vi "Prcess Data.vi"(8 "error in (no error)":errorcluster, 9 "Running":refnum<vi>, 10 "XY Plot":refnum<vi>, 11 "4way Lap":refnum<class "4way Lap.lvclass">) -> (0 "error out":errorcluster, 3 "4way Lap out":refnum<class "4way Lap.lvclass">)   [LabVIEW 2025, in "Flow Grind.lvlib" / "4way Lap.lvclass"]
uses:
  4way Lap.lvclass
  4way Lap.lvclass/4way Lap.ctl
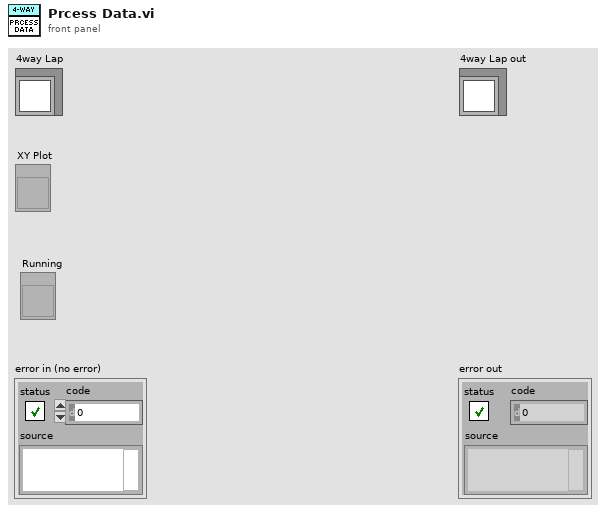
[diagram p1: front panel]
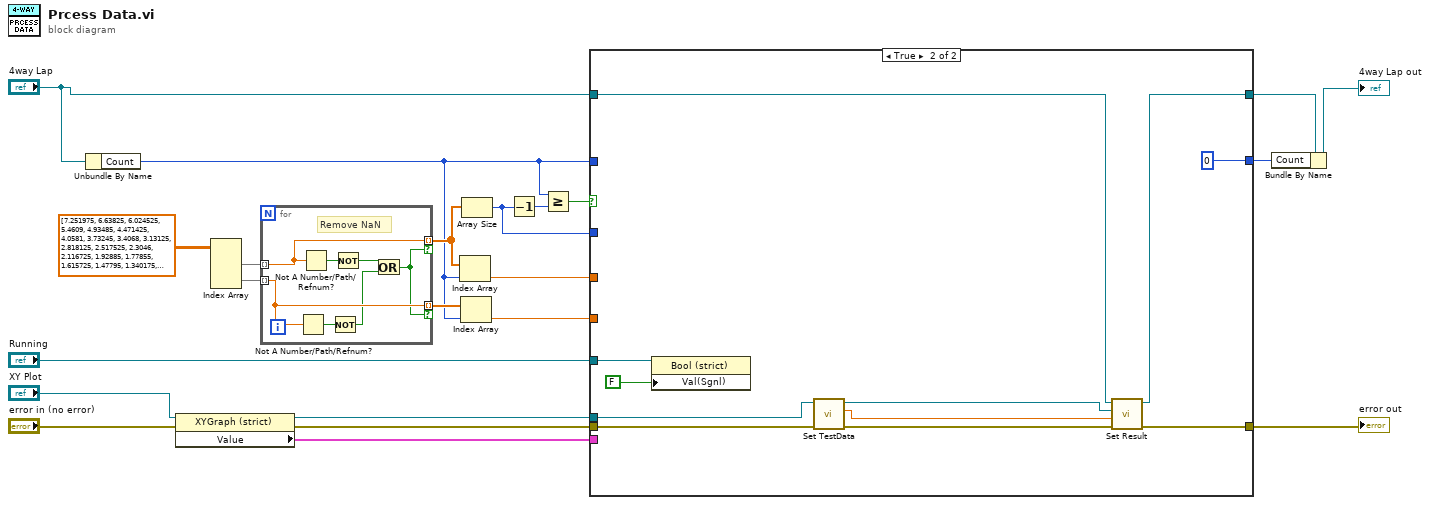
[diagram p0: block diagram]
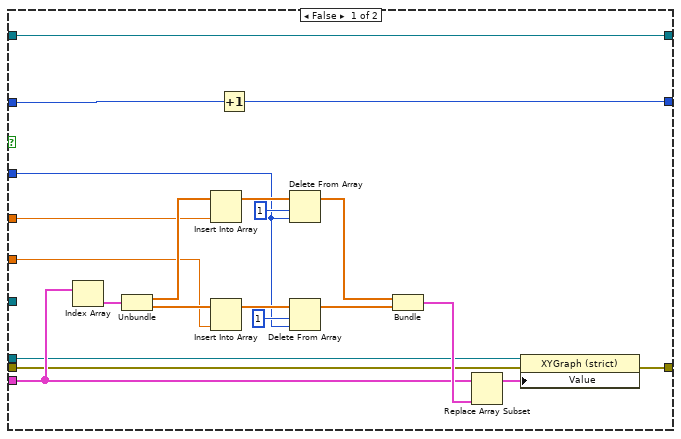
[diagram p2: hidden frame]
diagram:
  n1 = Unbundle By Name("4way Lap") -> ("Count"=w7:i32)
  n2 = property class="XYGraph (strict)"(reference="XY Plot", error in="error in (no error)") -> (reference out=w8:refnum<vi>, error out=w12:errorcluster, "Value"=w11:cluster{dbl[], dbl[]}[])
  n3 = Index Array(array=dbl[][] [[7.251975, 6.63825, 6.024525, 5.4609, 4.93485, 4.471425, 4.0581, 3.73245, 3.4068, 3.13125, 2.818125, 2.517525, 2.3046, 2.116725, 1.92885, 1.77855, 1.615725, 1.47795, 1.340175, 1.214925, 1.089675, 0.97695, 0.9018, 0.839175, 0.764025, 0.67635, 0.588675, 0.488475, 0.338175, 0.212925, 0.112725, -0.02505, -0.187875, -0.3507, -0.501, -0.62625, -0.7515, -0.864225, -0.97695, -1.0521, -1.1523, -1.27755, -1.415325, -1.490475, -1.62825, -1.8036, -1.9539, -2.1042, -2.241975, -2.4048, -2.592675, -2.768025, -2.9058, -3.08115, -3.269025, -3.469425, -3.694875, -3.920325, -4.13325, -4.38375, -4.696875, -4.98495, -5.298075, -5.648775, -5.9118, -6.224925, -6.550575, -6.951375], [-7.3443925, -6.7187476, -6.0917533, -5.5040949, -4.9617892, -4.4653641, -4.0162001, -3.6573409, -3.2980257, -2.9632382, -2.6025131, -2.270966, -2.0078164, -1.7655689, -1.539595, -1.3437553, -1.1485939, -0.9946363, -0.8398073, -0.7050944, -0.5807032, -0.4853256, -0.4206664, -0.3716988, -0.3245471, -0.2785864, -0.2304891, -0.1855597, -0.1344379, -0.0956821, -0.0690573, -0.03537, 0.0020509, 0.0484327, 0.098744, 0.1434598, 0.1871273, 0.2294166, 0.2676967, 0.2868859, 0.324321, 0.3887973, 0.4749279, 0.5426915, 0.6730592, 0.874013, 1.0799028, 1.29337, 1.5099154, 1.7484447, 2.0206898, 2.2772429, 2.4823522, 2.7123799, 2.9618931, 3.2030587, 3.4692113, 3.7435407, 4.0325076, 4.347976, 4.7024411, 5.0239845, 5.372376, 5.7437402, 6.0484042, 6.3833744, 6.7387807, 7.1376584], [0.0, 0.0, 0.0, 0.0, 0.0, 0.0, 0.0, 0.0, 0.0, 0.0, 0.0, 0.0, 0.0, 0.0, 0.0, 0.0, 0.0, 0.0, 0.0, 0.0, 0.0, 0.0, 0.0, 0.0, 0.0, 0.0, 0.0, 0.0, 0.0, 0.0, 0.0, 0.0, 0.0, 0.0, 0.0, 0.0, 0.0, 0.0, 0.0, 0.0, 0.0, 0.0, 0.0, 0.0, 0.0, 0.0, 0.0, 0.0, 0.0, 0.0, 0.0, 0.0, 0.0, 0.0, 0.0, 0.0, 0.0, 0.0, 0.0, 0.0, 0.0, 0.0, 0.0, 0.0, 0.0, 0.0, 0.0, 0.0], [0.0, 0.0, 0.0, 0.0, 0.0, 0.0, 0.0, 0.0, 0.0, 0.0, 0.0, 0.0, 0.0, 0.0, 0.0, 0.0, 0.0, 0.0, 0.0, 0.0, 0.0, 0.0, 0.0, 0.0, 0.0, 0.0, 0.0, 0.0, 0.0, 0.0, 0.0, 0.0, 0.0, 0.0, 0.0, 0.0, 0.0, 0.0, 0.0, 0.0, 0.0, 0.0, 0.0, 0.0, 0.0, 0.0, 0.0, 0.0, 0.0, 0.0, 0.0, 0.0, 0.0, 0.0, 0.0, 0.0, 0.0, 0.0, 0.0, 0.0, 0.0, 0.0, 0.0, 0.0, 0.0, 0.0, 0.0, 0.0]] ("array1")) -> (element #1=w22:dbl[], element #2=w21:dbl[])  [unwired: 4 in]
  n4 = for {
    tunnel: w22 -> [w29] mode=indexing
    tunnel: w21 -> [w26] mode=indexing
    tunnel: [w29] -> w18 mode=indexing if=w23
    tunnel: [w26] -> w20 mode=indexing if=w23
    # "Remove NaN"
    n5 = Not A Number/Path/Refnum?(number/path/refnum=w26) -> (NaN/Path/Refnum?=w27:bool)
    n6 = Not A Number/Path/Refnum?(number/path/refnum=w29) -> (NaN/Path/Refnum?=w28:bool)
    n7 = Not(x=w27) -> (.not. x?=w25:bool)
    n8 = Not(x=w28) -> (.not. x?=w24:bool)
    n9 = Or(x=w24, y=w25) -> (x .or. y?=w23:bool)
  }
  n10 = Index Array(array=w18, index=w7) -> (element=w16:dbl)
  n11 = Index Array(array=w20, index=w7) -> (element=w15:dbl)
  n12 = Array Size(array=w18) -> (size(s)=w5:i32)
  n13 = Decrement(x=w5) -> (x-1=w19:i32)
  n14 = Greater Or Equal?(x=w7, y=w19) -> (x >= y?=w17:bool)
  n15 = case shown="True" w17 {
    tunnel: w16 -> [w38 _]
    tunnel: w15 -> [w39 _]
    tunnel: w12 -> [w33 w60]
    tunnel: w11 -> [w40 _]
    tunnel: [w37 0] -> w9
    tunnel: w8 -> [w34 w55]
    tunnel: w7 -> [w36 _]
    tunnel: "Running" -> [_ w59]
    tunnel: w5 -> [w35 _]
    tunnel: [w31 w56] -> w4
    tunnel: "4way Lap" -> [w30 w52]
    tunnel: [w30 w51] -> w1
    frame False {
      n16 = Index Array(array=w40) -> (element=w49:cluster{dbl[], dbl[]})  [unwired: 1 in]
      n17 = Unbundle(w49) -> (w47:dbl[], w48:dbl[])
      n18 = Insert Into Array(array=w47, new element=w38) -> (w44:dbl[])  [unwired: 1 in]
      n19 = Insert Into Array(array=w48, new element=w39) -> (w45:dbl[])  [unwired: 1 in]
      n20 = Increment(x=w36) -> (x+1=w37:i32)
      n21 = Delete From Array(array=w44, length=1, index=w35) -> (array with subset deleted=w42:dbl[])  [unwired: 1 out]
      n22 = Delete From Array(array=w45, length=1, index=w35) -> (array with subset deleted=w41:dbl[])  [unwired: 1 out]
      n23 = Bundle(w42, w41) -> (w50:cluster{dbl[], dbl[]})  [unwired: 1 in]
      n24 = Replace Array Subset(array=w40, new element=w50) -> (w32:cluster{dbl[], dbl[]}[])  [unwired: 1 in]
      n25 = property class="XYGraph (strict)"(reference=w34, error in=w33, "Value"=w32) -> (error out=w31:errorcluster)  [unwired: 1 out]
    }
    frame True {
      n26 = property class="Bool (strict)"(reference=w59, "Val(Sgnl)"=FALSE ("Value (Signaling)")) -> ()  [unwired: 1 in, 2 out]
      n27 = call "Set TestData.vi"("error in (no error)"=w60, "Main"=w55) -> ("error out"=w57:errorcluster, "dS"=w53:dbl, "XY Plot out"=w54:refnum<vi>)  [unwired: 7 in]
      n28 = call "Set Result.vi"("error in (no error)"=w57, "dS"=w53, "XY Plot"=w54, "4way Lap in"=w52) -> ("error out"=w56:errorcluster, "4way Lap out"=w51:refnum<class "4way Lap.lvclass">)  [unwired: 6 in]
    }
  }
  "error out" <- w4
  n29 = Bundle By Name(cluster=w1, "Count"=w9) -> (→"4way Lap out":refnum<class "4way Lap.lvclass">)
